vi "任意波形绘制.vi"(8 "曲线设置":T2, 10 "历史数据":T3[](array[typedef]), 11 "映射方式":T1) -> (0 "曲线属性":cluster{"曲线名":string, "曲线颜色":u32, "线条宽度":u8}[](array[cluster]), 3 "XY图":cluster{"数据":dbl[], "数据":dbl[]}[](array[cluster]))   [LabVIEW 2020, in "数据显示.xctl"]
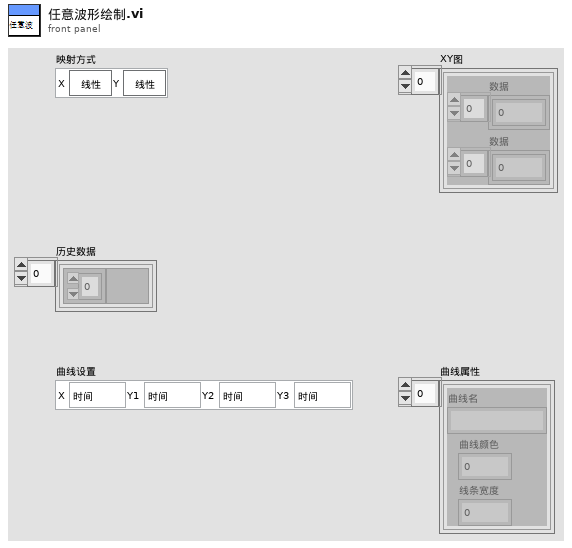
[diagram p1: front panel]
types:
  T1 = typedef "数据显示.xctl/映射方式.ctl" = cluster{"X":bool, "Y":bool}
  T2 = typedef "数据显示.xctl/曲线设置.ctl" = cluster{"X":enum16{"时间", "设置电压", "读取电流", "读取电压"}, "Y1":enum16{"时间", "设置电压", "读取电流", "读取电压"}, "Y2":enum16{"时间", "设置电压", "读取电流", "读取电压", "无"}, "Y3":enum16{"时间", "设置电压", "读取电流", "读取电压", "无"}}
  T3 = typedef "数据显示.xctl/波形数据定义.ctl" = cluster{"波形":dbl[][], "属性":variant}
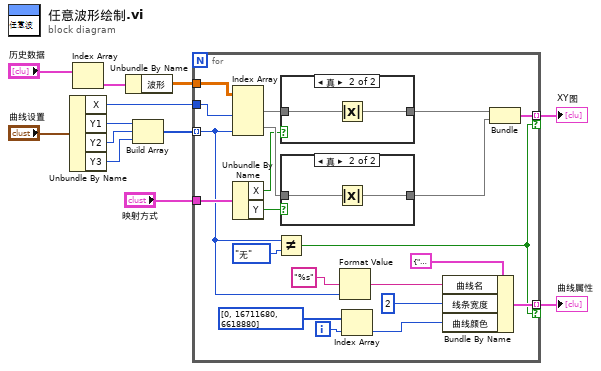
[diagram p0: block diagram]
diagram:
  n1 = Unbundle By Name("曲线设置") -> ("X"=w3:enum16{"时间", "设置电压", "读取电流", "读取电压"}, "Y1"=w4:enum16{"时间", "设置电压", "读取电流", "读取电压"}, "Y2"=w5:enum16{"时间", "设置电压", "读取电流", "读取电压", "无"}, "Y3"=w6:enum16{"时间", "设置电压", "读取电流", "读取电压", "无"})
  n2 = Index Array(array="历史数据") -> (element=w9:T3)  [unwired: 1 in]
  n3 = Unbundle By Name(w9) -> ("波形"=w10:dbl[][])
  n4 = Build Array(w4, w5, w6) -> (w7:enum16{"时间", "设置电压", "读取电流", "读取电压", "无"}[])
  n5 = for {
    tunnel: w10 -> [w33]
    tunnel: w3 -> [w14]
    tunnel: w7 -> [w13] mode=indexing
    tunnel: "映射方式" -> [w32]
    tunnel: [w24] -> w12 mode=indexing if=w20
    tunnel: [w23] -> w11 mode=indexing if=w20
    i -> [w18]
    n6 = Index Array(array=w33, index (col) #1=w14, index (col) #2=w13) -> (element #1=w31:dbl[], element #2=w30:dbl[])  [unwired: 2 in]
    n7 = Unbundle By Name(w32) -> ("X"=w27:bool, "Y"=w26:bool)
    n8 = Not Equal?(x=w13, y=enum16{"时间", "设置电压", "读取电流", "读取电压", "无"}."无") -> (x != y?=w20:bool)
    n9 = case shown="真" w27 {
      tunnel: w31 -> [w37 w39]
      tunnel: [w37 w38] -> w29
      frame False {
      }
      frame True {
        n10 = Absolute Value(x=w39) -> (abs(x)=w38:dbl[])
      }
    }
    n11 = case shown="真" w26 {
      tunnel: w30 -> [w34 w36]
      tunnel: [w34 w35] -> w28
      frame False {
      }
      frame True {
        n12 = Absolute Value(x=w36) -> (abs(x)=w35:dbl[])
      }
    }
    n13 = Format Value(format string="%s" ("格式字符串"), value (0)=w13) -> (output string=w15:string)  [unwired: 1 in]
    n14 = Index Array(array=u32[] [0, 16711680, 6618880], index=w18) -> (element=w17:u32)
    n15 = Bundle By Name(cluster=cluster{"曲线名":string, "曲线颜色":u32, "线条宽度":u8} {"曲线名"="", "曲线颜色"=0, "线条宽度"=0} ("曲线属性"), "曲线名"=w15, "线条宽度"=u8 2, "曲线颜色"=w17) -> (w23:cluster{"曲线名":string, "曲线颜色":u32, "线条宽度":u8})
    n16 = Bundle("波形"=w29, "波形"=w28) -> (w24:cluster{"波形":dbl[], "波形":dbl[]})  [unwired: 1 in]
  }
  "XY图" <- w12
  "曲线属性" <- w11
